vi "query Operation Band.vi"(8 "error in (no error)":errorcluster, 11 "LTE in":refnum<class "LTE.lvclass">) -> (0 "error out":errorcluster, 2 "Operation Band":u32, 3 "LTE out":refnum<class "LTE.lvclass">)   [LabVIEW 2023, in "ANRITSU Call Box.lvlib" / "LTE.lvclass"]
uses:
  LTE.lvclass
  LTE.lvclass/LTE.ctl
  ANRITSU Call Box.lvlib
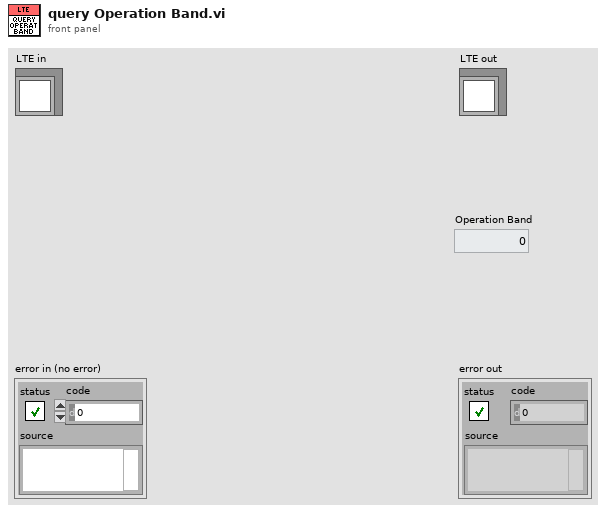
[diagram p1: front panel]
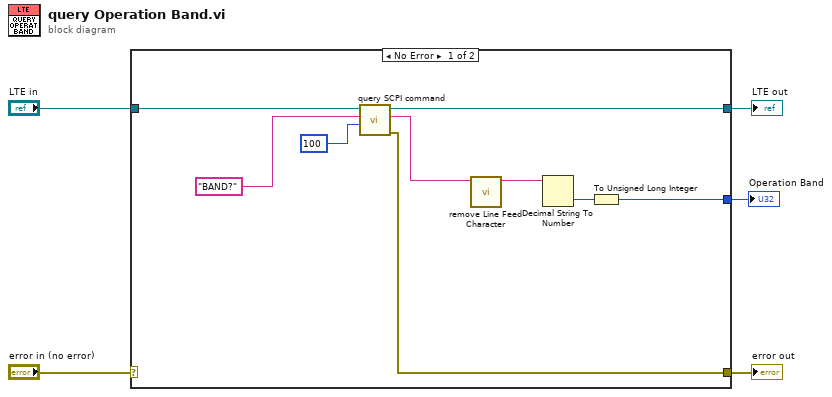
[diagram p0: block diagram]
diagram:
  n1 = case shown="No Error" "error in (no error)" {
    selector: "error in (no error)" -> [_ w16]
    tunnel: [w7 w16] -> w4
    tunnel: [w8 w15] -> w2
    tunnel: "LTE in" -> [w14 w15]
    tunnel: [w6 _] -> w1
    frame No Error {
      n2 = call "query SCPI command.vi"("Read Buffer Length"=u32 100, "SCPI Command"="BAND?", "LTE in"=w14) -> ("error out"=w7:errorcluster, "Read Buffer String"=w11:string, "LTE out"=w8:refnum<class "LTE.lvclass">)  [unwired: 6 in]
      n3 = call "remove Line Feed Character.vi"("Query String"=w11) -> ("Line Feed Removed String"=w9:string)  [unwired: 9 in, 1 out]
      n4 = Decimal String To Number(string=w9) -> (number=w10:i32)  [unwired: 2 in, 1 out]
      n5 = To Unsigned Long Integer(number=w10) -> (unsigned 32bit integer=w6:u32)
    }
    frame Error {
    }
  }
  "error out" <- w4
  "LTE out" <- w2
  "Operation Band" <- w1
